vi "JOYSTICK.vi"() -> ()   [LabVIEW 2020]
uses:
  <vilib>/Instr/_visa.llb/VISA Configure Serial Port (Instr).vi
  <vilib>/Utility/inputDevices.llb/joystickAcquire.vi
  <vilib>/Utility/inputDevices.llb/closeJoystick.vi
panel:
  out "concatenated string":string
  in  "VISA resource name":refnum<visa-resource-name>
  out "DIRRECION":dbl(knob) scale=-90.0..90.0
  out "VELOCIDAD":dbl(knob) scale=0.0..100.0
  out "VERDE":bool
  out "ROJO":bool
  out "Z axis":i32
  out "X axis rotation":i32
  in  "stop":bool
  in  "device index":i32
  out "joystick info":T1(array[cluster])
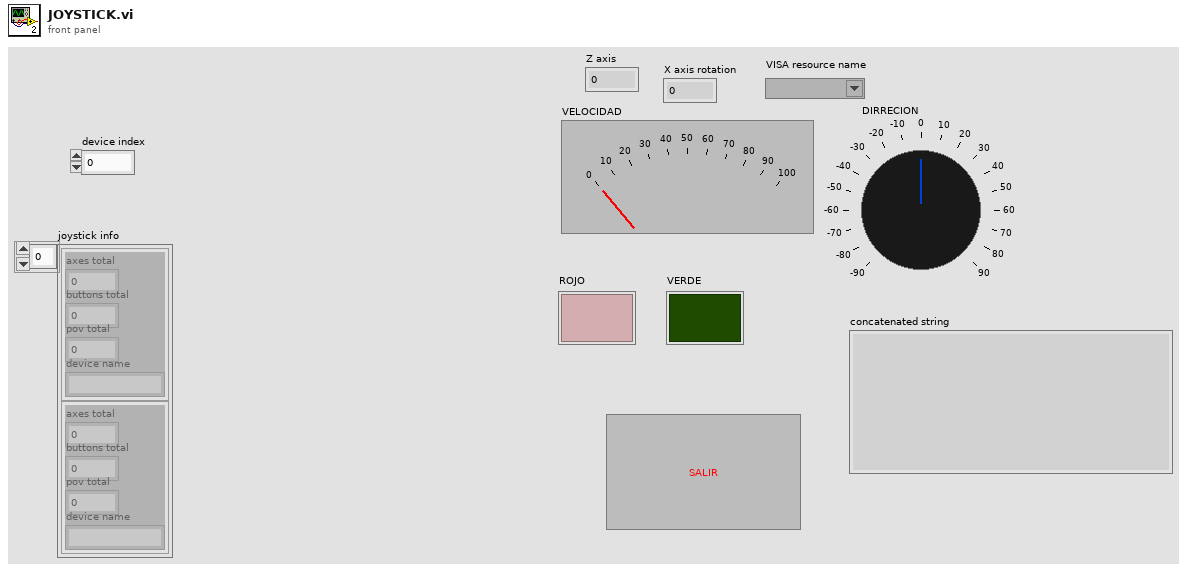
[diagram p1: front panel]
types:
  T1 = cluster{"axes total":u32, "buttons total":u32, "pov total":u32, "device name":string}[]
  T2 = cluster{"X axis":i32, "Y axis":i32, "Z axis":i32, "X axis rotation":i32, "Y axis rotation":i32, "Z axis rotation":i32, "U axis":i32, "V axis":i32}
  T3 = cluster{"button 1":bool, "button 2":bool, "button 3":bool, "button 4":bool, "button 5":bool, "button 6":bool, "button 7":bool, "button 8":bool, "button 9":bool, "button 10":bool, "button 11":bool, "button 12":bool, "button 13":bool, "button 14":bool, "button 15":bool, "button 16":bool, "button 17":bool, "button 18":bool, "button 19":bool, "button 20":bool, "button 21":bool, "button 22":bool, "button 23":bool, "button 24":bool, "button 25":bool, "button 26":bool, "button 27":bool, "button 28":bool, "button 29":bool, "button 30":bool, "button 31":bool, "button 32":bool}
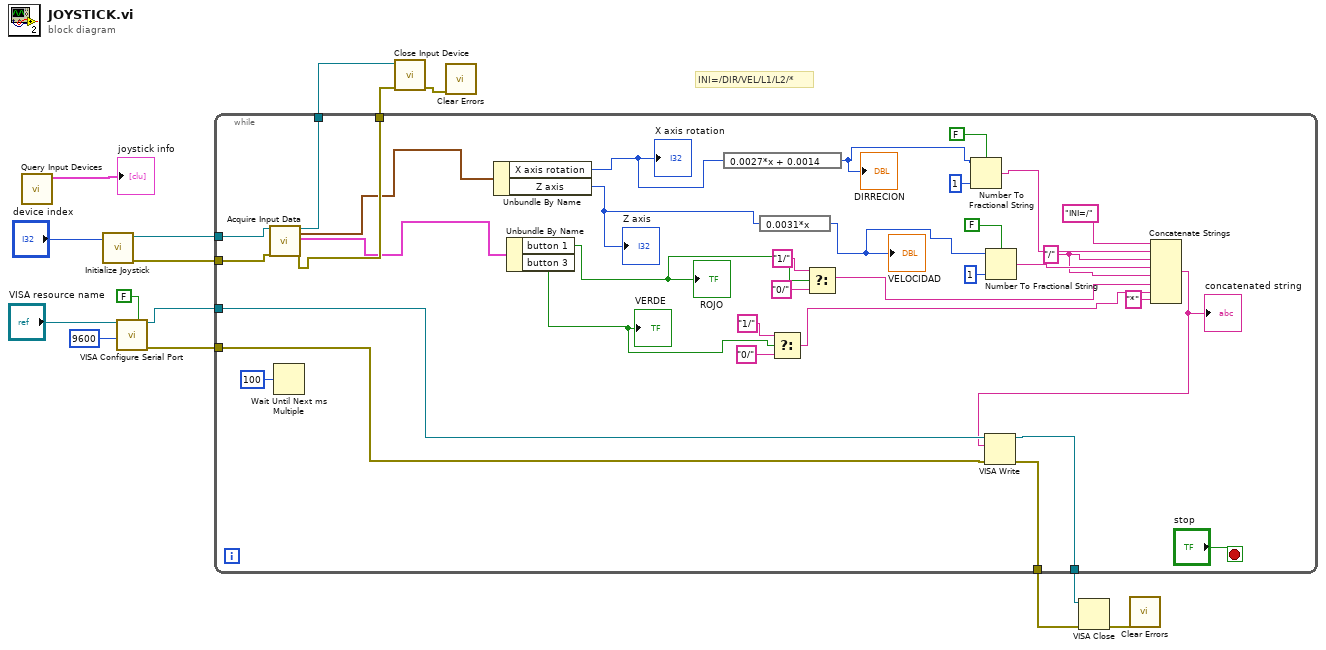
[diagram p0: block diagram]
diagram:
  # "INI=/DIR/VEL/L1/L2/*"
  n1 = call <vilib>:"Query Input Devices.vi"() -> ("joystick info"=→"joystick info":T1)  [unwired: 8 in, 3 out]
  n2 = call <vilib>:"Initialize Joystick.vi"("device index"="device index") -> ("error out"=w12:errorcluster, "device ID"=w13:refnum<k1>)  [unwired: 9 in]
  n3 = call-poly "VISA Configure Serial Port"("VISA resource name"="VISA resource name", "Enable Termination\nChar (T)"=FALSE ("Enable Termination\nChar (T)"), "baud rate (9600)"=u32 9600) -> ("VISA resource name out"=w2:refnum<visa-resource-name>, "error out"=w1:errorcluster)  [unwired: 11 in]
  n4 = while {
    tunnel: w13 -> [w48]
    tunnel: w12 -> [w47]
    tunnel: [w46] -> w11
    tunnel: [w45] -> w10
    tunnel: [w39] -> w4
    tunnel: [w38] -> w3
    tunnel: w2 -> [w37]
    tunnel: w1 -> [w36]
    stop <- "stop" stop-if-true
    w20 = "/" ("string")
    n5 = call-poly <vilib>:"Acquire Input Data.vi"("device ID"=w48, "error in (no error)"=w47) -> ("device ID"=w45:refnum<k1>, "axis info"=w44:T2, "button info"=w43:T3, "error out"=w46:errorcluster)  [unwired: 13 in, 1 out]
    n6 = Wait Until Next ms Multiple(millisecond multiple=u32 100) -> ()  [unwired: 1 out]
    n7 = Unbundle By Name(w44) -> ("X axis rotation"=w42:i32, "Z axis"=w41:i32)
    "X axis rotation" <- w42
    "Z axis" <- w41
    n8 = Unbundle By Name(w43) -> ("button 1"=w29:bool, "button 3"=w24:bool)
    "VERDE" <- w24
    "ROJO" <- w29
    n9 = expression code="0.0027*x + 0.0014"(w42) -> (w35:i32)
    "DIRRECION" <- w35
    n10 = expression code="0.0031*x"(w41) -> (w30:i32)
    "VELOCIDAD" <- w30
    n11 = Select(t="1/", s=w24, f="0/") -> (s? t:f=w18:string)
    n12 = Select(t="1/", s=w29, f="0/") -> (s? t:f=w19:string)
    n13 = Number To Fractional String(use system decimal point (T)=FALSE, number=w35, precision (6)=i16 1) -> (F-format string=w22:string)  [unwired: 1 in]
    n14 = Number To Fractional String(use system decimal point (T)=FALSE, number=w30, precision (6)=i16 1) -> (F-format string=w21:string)  [unwired: 1 in]
    n15 = Concatenate Strings("INI=/" ("string"), w22, w20, w21, w20, w19, w18, "*" ("string")) -> (w16:string)
    "concatenated string" <- w16
    n16 = VISA Write(VISA resource name=w37, write buffer=w16, error in (no error)=w36) -> (VISA resource name out=w39:refnum<visa-resource-name>, error out=w38:errorcluster)  [unwired: 1 out]
  }
  n17 = call-poly <vilib>:"Close Input Device.vi"("error in (no error)"=w11, "device ID"=w10) -> ("error out"=w9:errorcluster)  [unwired: 8 in]
  n18 = call <vilib>:"Clear Errors.vi"("error in (no error)"=w9) -> ()  [unwired: 5 in, 2 out]
  n19 = VISA Close(VISA resource name=w4, error in (no error)=w3) -> (error out=w5:errorcluster)
  n20 = call <vilib>:"Clear Errors.vi"("error in (no error)"=w5) -> ()  [unwired: 5 in, 2 out]
